vi "ConvertToStandJSON.vi"(8 "error in (no error)":errorcluster, 11 "caps":string) -> (0 "error out":errorcluster, 3 "json caps":string)   [LabVIEW 2017, in "Paser.lvlib"]
uses:
  Paser.lvlib
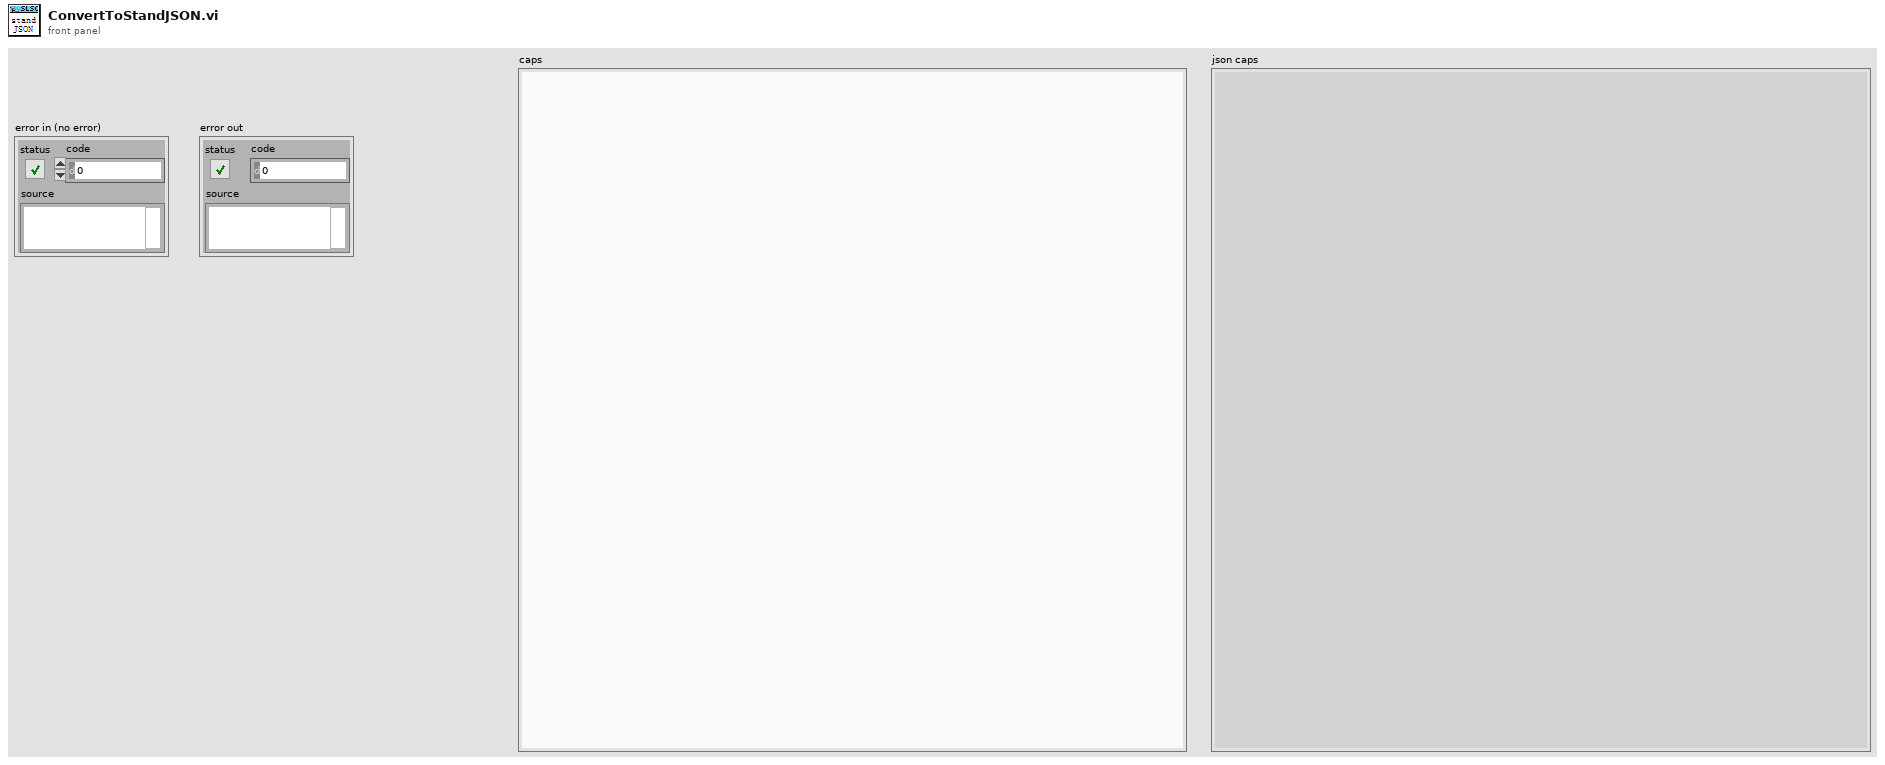
[diagram p1: front panel]
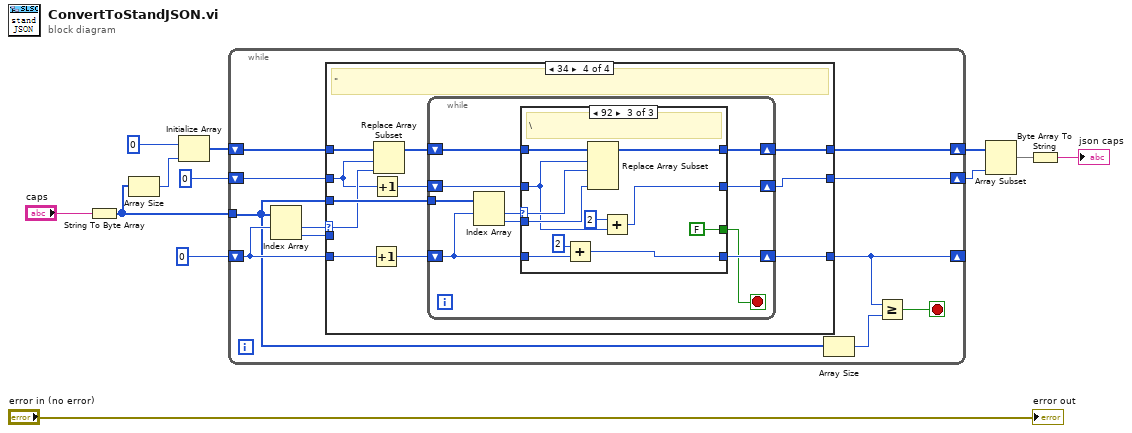
[diagram p0: block diagram]
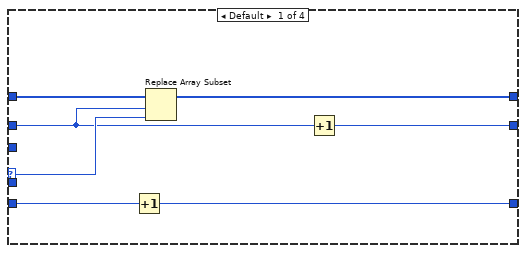
[diagram p2: hidden frame]
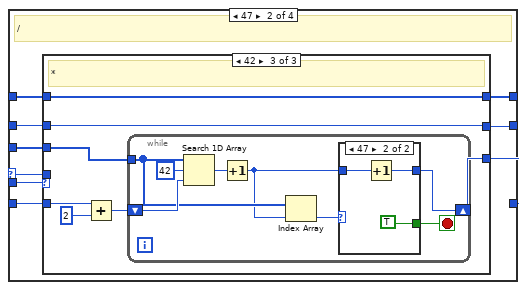
[diagram p3: hidden frame]
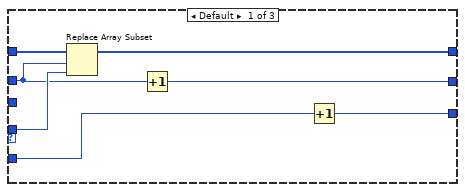
[diagram p4: hidden frame]
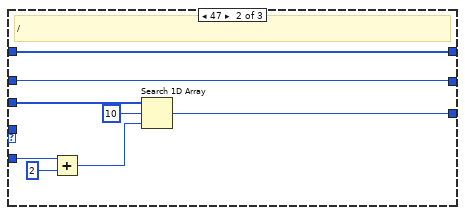
[diagram p5: hidden frame]
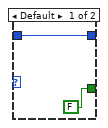
[diagram p6: hidden frame]
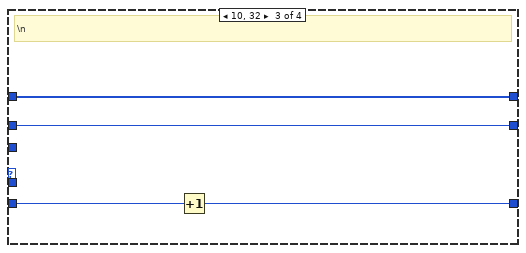
[diagram p7: hidden frame]
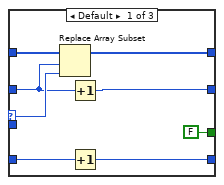
[diagram p8: hidden frame]
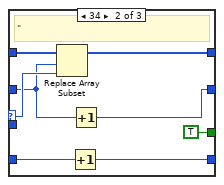
[diagram p9: hidden frame]
diagram:
  n1 = String To Byte Array(string="caps") -> (unsigned byte array=w9:u8[])
  n2 = Array Size(array=w9) -> (size(s)=w8:i32)
  n3 = Initialize Array(u8 0, w8) -> (w10:u8[])
  n4 = while {
    tunnel: w9 -> [w18]
    shift-right: [w15] -> _
    shift-left: 0 -> [w21]
    shift-right: [w13] -> w4
    shift-left: 0 -> [w14]
    shift-right: [w19] -> w5
    shift-left: w10 -> [w20]
    stop <- w17 stop-if-true
    n5 = Index Array(array=w18, index #1=w21) -> (element #1=w23:u8, element #2=w22:u8)  [unwired: 1 in]
    n6 = case shown="34" w23 {
      selector: w23 -> [w26 w35 _ w82]
      tunnel: w22 -> [_ w39 _ _]
      tunnel: w21 -> [w29 w38 w77 w88]
      tunnel: w18 -> [_ w37 _ w87]
      tunnel: [w28 w33 w75 w83] -> w15
      tunnel: w20 -> [w30 w36 w78 w89]
      tunnel: [w27 w34 w78 w84] -> w19
      tunnel: w14 -> [w25 w32 w76 w81]
      tunnel: [w24 w31 w76 w79] -> w13
      frame Default {
        n7 = Increment(x=w29) -> (x+1=w28:i32)
        n8 = Replace Array Subset(array=w30, new element=w26, index=w25) -> (w27:u8[])
        n9 = Increment(x=w25) -> (x+1=w24:i32)
      }
      frame 47 {
        # "/"
        n10 = case shown="42" w39 {
          tunnel: w38 -> [w44 w54 w61]
          tunnel: w37 -> [_ w52 w57]
          tunnel: [w43 w48 w56] -> w33
          tunnel: w36 -> [w46 w49 w59]
          tunnel: w35 -> [w42 _ _]
          tunnel: [w45 w49 w59] -> w34
          tunnel: w32 -> [w41 w47 w55]
          tunnel: [w40 w47 w55] -> w31
          frame Default {
            n11 = Replace Array Subset(array=w46, new element=w42, index=w41) -> (w45:u8[])
            n12 = Increment(x=w41) -> (x+1=w40:i32)
            n13 = Increment(x=w44) -> (x+1=w43:i32)
          }
          frame 47 {
            # "/"
            n14 = Add(x=w54, y=2) -> (x+y=w51:i32)
            n15 = Search 1D Array(1D array=w52, element=u8 10, start index (0)=w51) -> (index of element=w48:i32)
          }
          frame 42 {
            # "*"
            n16 = Add(x=w61, y=2) -> (x+y=w58:i32)
            n17 = while {
              tunnel: w57 -> [w66]
              shift-right: [w62] -> w56
              shift-left: w58 -> [w69]
              stop <- w64 stop-if-true
              n18 = Search 1D Array(1D array=w66, element=u8 42, start index (0)=w69) -> (index of element=w67:i32)
              n19 = Increment(x=w67) -> (x+1=w63:i32)
              n20 = Index Array(array=w66, index=w63) -> (element=w65:u8)
              n21 = case shown="47" w65 {
                tunnel: [FALSE TRUE] -> w64
                tunnel: w63 -> [w71 w73]
                tunnel: [w71 w72] -> w62
                frame Default {
                }
                frame 47 {
                  n22 = Increment(x=w73) -> (x+1=w72:i32)
                }
              }
            }
          }
        }
      }
      frame 10, 32 {
        # "\\n"
        n23 = Increment(x=w77) -> (x+1=w75:i32)
      }
      frame 34 {
        # "\""
        n24 = Increment(x=w88) -> (x+1=w86:i32)
        n25 = Increment(x=w81) -> (x+1=w80:i32)
        n26 = Replace Array Subset(array=w89, new element=w82, index=w81) -> (w85:u8[])
        n27 = while {
          tunnel: w87 -> [w99]
          shift-right: [w93] -> w83
          shift-left: w86 -> [w94]
          shift-right: [w95] -> w84
          shift-left: w85 -> [w97]
          shift-right: [w90] -> w79
          shift-left: w80 -> [w91]
          stop <- w92 stop-if-true
          n28 = Index Array(array=w99, index #1=w94) -> (element #1=w98:u8, element #2=w96:u8)  [unwired: 1 in]
          n29 = case shown="92" w98 {
            selector: w98 -> [w102 w110 w119]
            tunnel: w97 -> [w107 w115 w126]
            tunnel: w96 -> [_ _ w120]
            tunnel: [w106 w114 w125] -> w95
            tunnel: w94 -> [w105 w113 w124]
            tunnel: [w104 w112 w122] -> w93
            tunnel: [FALSE TRUE FALSE] -> w92
            tunnel: w91 -> [w101 w109 w117]
            tunnel: [w100 w108 w116] -> w90
            frame Default {
              n30 = Replace Array Subset(array=w107, new element=w102, index=w101) -> (w106:u8[])
              n31 = Increment(x=w101) -> (x+1=w100:i32)
              n32 = Increment(x=w105) -> (x+1=w104:i32)
            }
            frame 34 {
              # "\""
              n33 = Replace Array Subset(array=w115, new element=w110, index=w109) -> (w114:u8[])
              n34 = Increment(x=w113) -> (x+1=w112:i32)
              n35 = Increment(x=w109) -> (x+1=w108:i32)
            }
            frame 92 {
              # "\\"
              n36 = Add(x=2, y=w124) -> (x+y=w122:i32)
              n37 = Replace Array Subset(array=w126, new element #1=w119, index #1=w117, new element #2=w120) -> (w125:u8[])  [unwired: 1 in]
              n38 = Add(x=2, y=w117) -> (x+y=w116:i32)
            }
          }
        }
      }
    }
    n39 = Array Size(array=w18) -> (size(s)=w16:i32)
    n40 = Greater Or Equal?(x=w15, y=w16) -> (x >= y?=w17:bool)
  }
  n41 = Array Subset(array=w5, length=w4) -> (w3:u8[])  [unwired: 1 in]
  n42 = Byte Array To String(unsigned byte array=w3) -> (string=→"json caps":string)
  "error out" <- "error in (no error)"
